vi "总控程序 _2026.vi"() -> ()   [LabVIEW 2026]
uses:
  Supports/CSM Names.ctl
  Supports/sPanel Data.ctl
  <userlib>/_NEVSTOP/Communicable State Machine(CSM)/_Polymophic/CSM - Filter Duplicated Lines.vi
  76f8fc9d-696a-4ccc-8dd7-48bdb3d8b640.vi
  bb814cf8-2670-4bb2-81f9-09f44a02b01b.vi
  fcea05e1-ee31-4bad-8a55-4c21f91279eb.vi
  86c0e0eb-f419-4f98-b770-132e8c8a6837.vi
  4aaf4cac-01b3-4f48-b7c2-c419dc6ea011.vi
  6f23f83d-c4e9-4f99-a0e1-96770a8349f6.vi
  8f3727b1-d436-4491-a02b-c19b6576eb4a.vi
  3b795a98-2c3e-48b2-8c77-c6d72b6bb2f2.vi
  a3e68da9-8157-4524-98c0-5afabb5447f5.vi
  436c64fb-213b-48d1-93d7-30f6f7eef33b.vi
  86e951a0-9aaf-40ac-b60e-6206b3d1b492.vi
  <userlib>/_NEVSTOP/Communicable State Machine(CSM)/_Polymophic/CSM - Replace Marks in Messages.vi
  29ebbcbd-9bba-4aa0-9480-6c7032d08e2a.vi
  31245a41-a78f-4281-aa79-3581d5ea05b1.vi
  ac877760-a0f7-42e3-86ce-81130eb57136.vi
  bb062149-d510-40e2-9bfa-d104bbeea636.vi
  <userlib>/_NEVSTOP/Communicable State Machine(CSM)/AdvanceAPI/CSM - Compact Multiple States.vi
  <userlib>/_NEVSTOP/Communicable State Machine(CSM)/AdvanceAPI/CSM - Break Down Multiple States String.vi
  <userlib>/_NEVSTOP/Communicable State Machine(CSM)/_Shared/Remove Comments from Single-line.vi
  <userlib>/_NEVSTOP/Communicable State Machine(CSM)/_Shared/Split Single-line Message.vi
  <userlib>/_NEVSTOP/Communicable State Machine(CSM)/_Shared/Trim Single-line Text.vi
  <userlib>/_NEVSTOP/Communicable State Machine(CSM)/AdvanceAPI/CSM - Revert Arguments-Safe String.vi
  <userlib>/_NEVSTOP/Communicable State Machine(CSM)/AdvanceAPI/CSM - Make String Arguments Safe.vi
  <userlib>/_NEVSTOP/Communicable State Machine(CSM)/AdvanceAPI/CSM - Keywords.vi
  <userlib>/_NEVSTOP/Communicable State Machine(CSM)/addons/API-String-Arugments-Support/_Support/Data To API String Arguments.vi
  <userlib>/_NEVSTOP/Communicable State Machine(CSM)/addons/INI-Static-Variable-Support/_Support/instances/_CSM - Read File Logger Configuration - v1.0.vi
  <userlib>/_NEVSTOP/Communicable State Machine(CSM)/addons/API-String-Arugments-Support/_Support/Convert API String Arguments to Data(variant).vi
  <userlib>/_NEVSTOP/Communicable State Machine(CSM)/Communicable State Machine.lvlib
  <userlib>/_NEVSTOP/Communicable State Machine(CSM)/addons/MassData-Parameter/CSM MassData Parameter Support.lvlib
  <userlib>/_NEVSTOP/Communicable State Machine(CSM)/addons/INI-Static-Variable-Support/INI-Static-Variable-Support.lvlib
  <userlib>/_NEVSTOP/Communicable State Machine(CSM)/addons/Watchdog/CSM Watchdog.lvlib
  <userlib>/_NEVSTOP/Communicable State Machine(CSM)/addons/Logger/CSM File Logger.lvlib
panel:
  in  "DS1":bool
  in  "HM1":bool
  in  "MO2":bool
  in  "MO1":bool
  in  "ZO1":bool
  in  "PS2":bool
  in  "PS1":bool
  in  "WK2":bool
  in  "P3-C3开关":bool
  in  "P3-C2开关":bool
  in  "P2-C3开关":bool
  in  "P2-C2开关":bool
  in  "P1-C3开关":bool
  in  "P1-C2开关":bool
  in  "WK1":bool
  in  "TP2":bool
  in  "TP1":bool
  in  "OP3":bool
  in  "OP2":bool
  in  "OP1":bool
  in  "停止":bool
  in  "波形查看":T1(tab)
  in  "合并保存？":bool
  in  "温度数据保存文件-时间":string
  in  "CSM Name":string="CSM-Module"
  out "State History":string
  out "Error Occurred":errorcluster
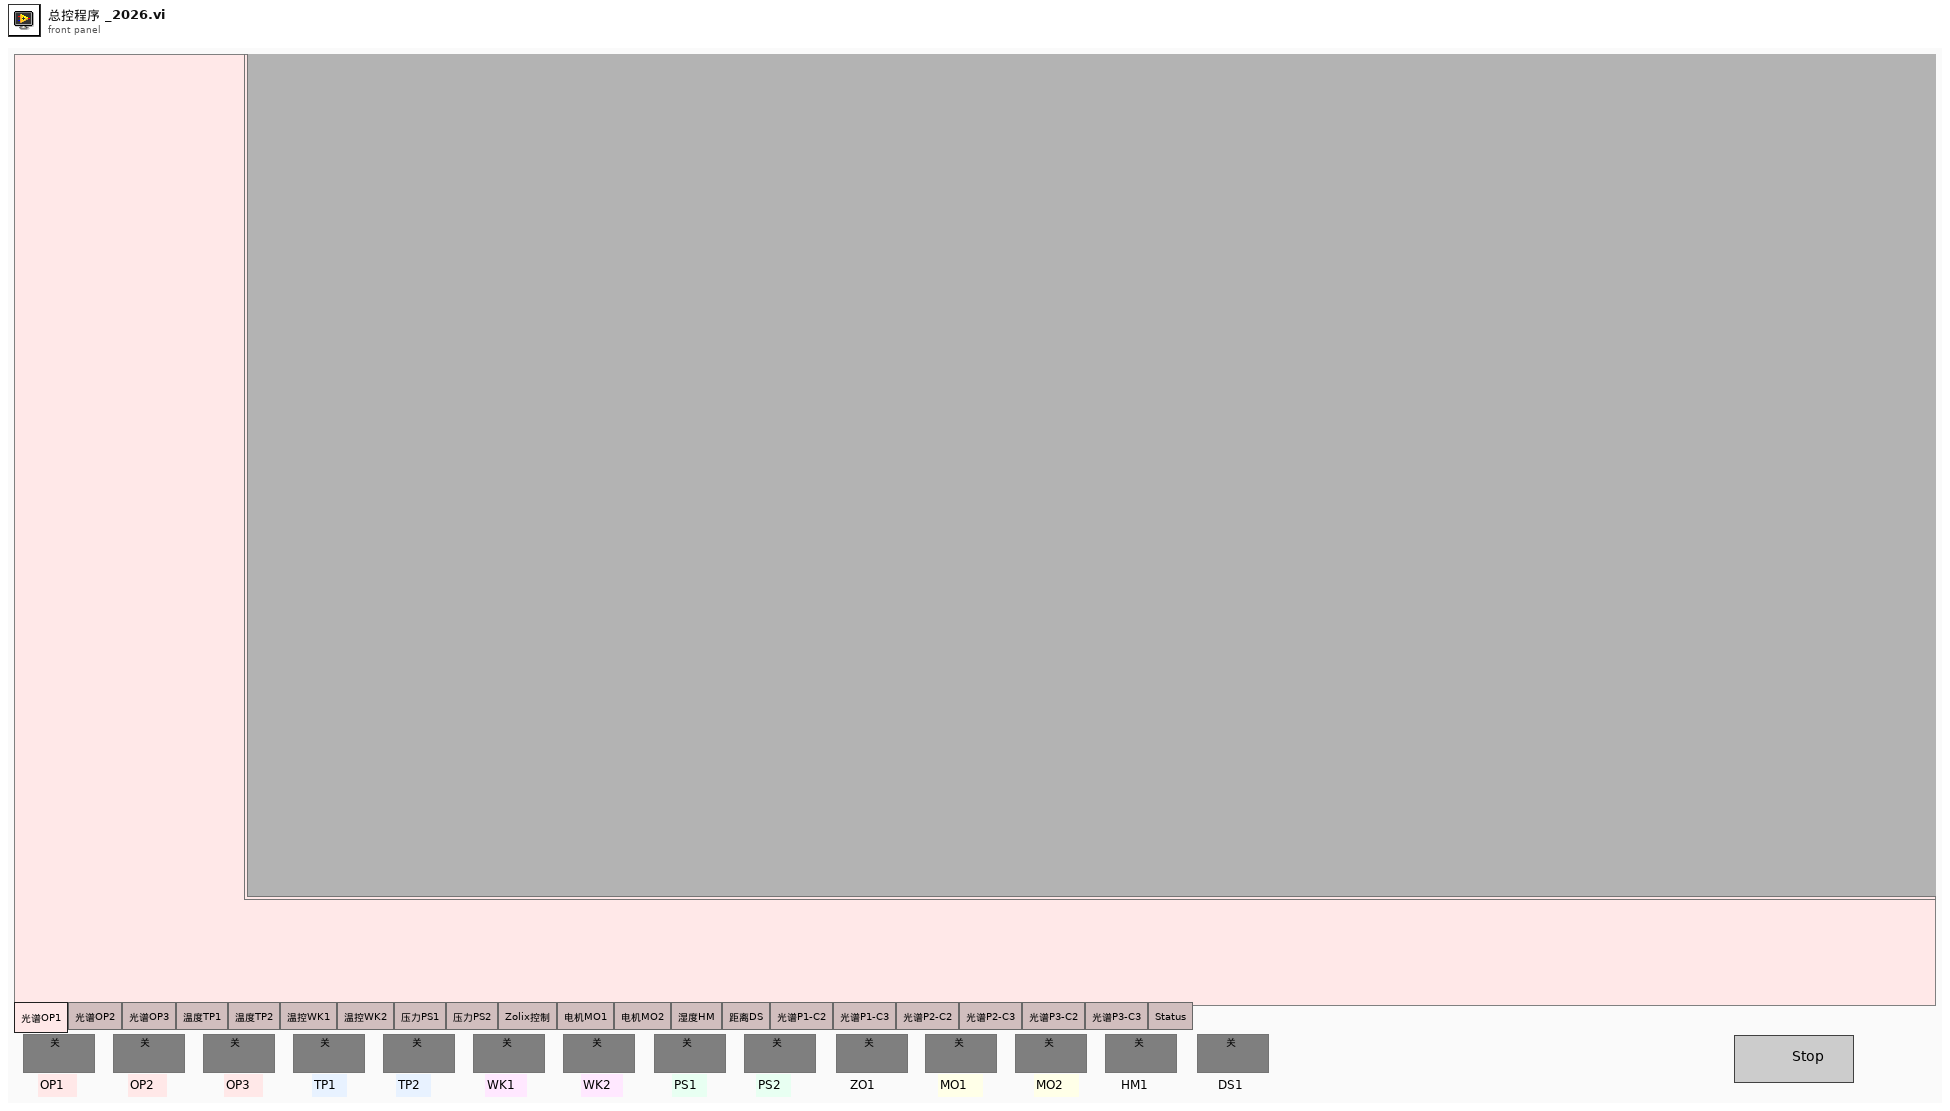
[diagram p1: front panel]
types:
  T1 = enum32{"光谱OP1", "光谱OP2", "光谱OP3", "温度TP1", "温度TP2", "温控WK1", "温控WK2", "压力PS1", "压力PS2", "Zolix控制", "电机MO1", "电机MO2", "湿度HM", "距离DS", "光谱P1-C2", "光谱P1-C3", "光谱P2-C2", "光谱P2-C3", "光谱P3-C2", "光谱P3-C3", "Status"}
  T2 = cluster{"Enable":bool, "Limit":cluster{"FileSize":i64, "FileNum":i32}, "Timestamp.Format":string, "AutoExit":bool}
  T3 = enum32{"Invalid", "Standard", "Closed", "Hidden", "Minimized", "Maximized"}
  T4 = enum32{"invalid app kind", "Development System", "Run Time System", "Student Edition", "Embedded LabVIEW", "Evaluation", "Custom"}
  T5 = typedef "sPanel Data.ctl" = cluster{"子面板":refnum<vi>, "程序引用":refnum<vi>, "CSM Name":string}
  T6 = typedef "温度保存信息.ctl" = cluster{"温度保存-时间":string, "合并保存？":bool, "保存路径":path, "Intervals":dbl}
  T7 = typedef "Communicable State Machine.lvlib/_CSM_Response Source Message.ctl" = cluster{"‘State":string, "’Arguments":string, "’Error":errorcluster}
  T8 = cluster{"Current VI Reference":refnum<vi>, "Close Panel on Exit?":bool}
  T9 = typedef "CSM Names.ctl" = string[]
  T10 = cluster{"Core":cluster{"Current VI Reference":refnum<vi>, "Close Panel on Exit?":bool}, "索引汇总":cluster{"子面板索引":refnum<vi>[], "程序索引":refnum<vi>[], "CSM Names":T9, "开关索引":refnum<vi>[]}, "Data Save":bool, "Stop":bool}
  T11 = cluster{"子面板索引":refnum<vi>[], "程序索引":refnum<vi>[], "CSM Names":T9, "开关索引":refnum<vi>[]}
  T12 = cluster{"子面板HM1":refnum<vi>, refnum<vi>, "CSM Name":string}
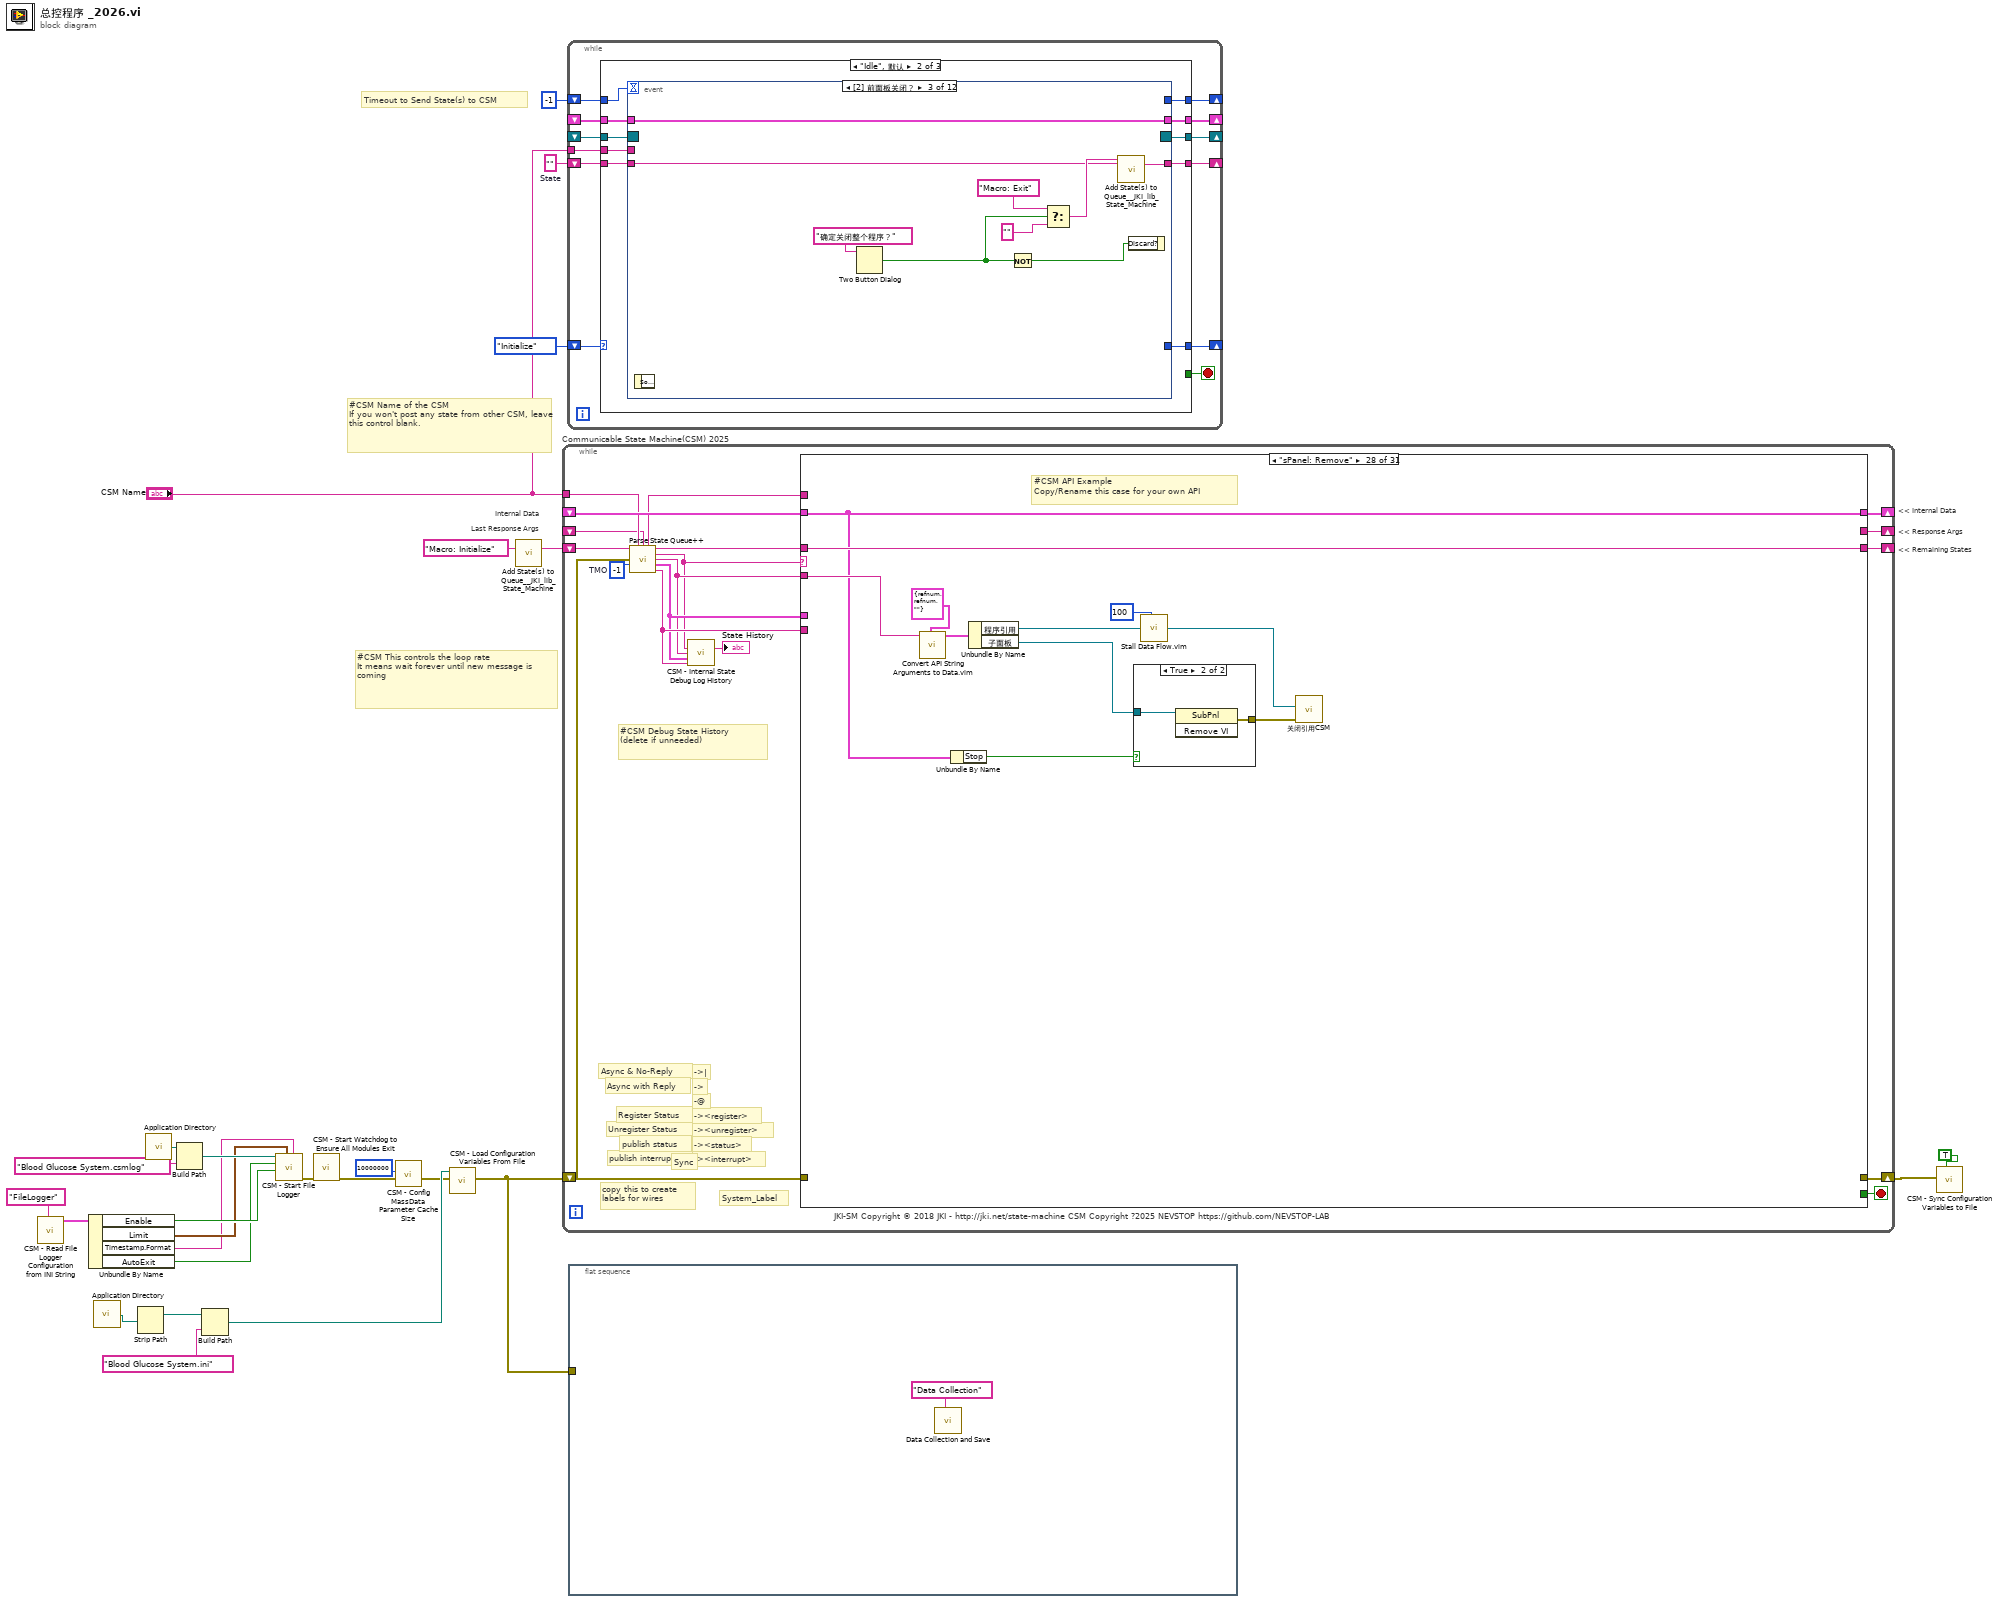
[diagram p0: block diagram]
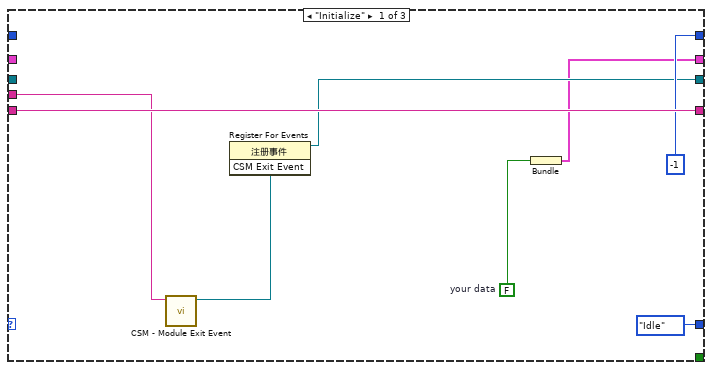
[diagram p2: hidden frame]
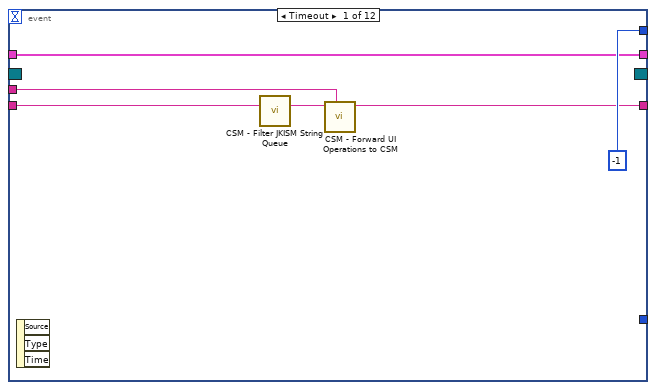
[diagram p3: hidden frame]
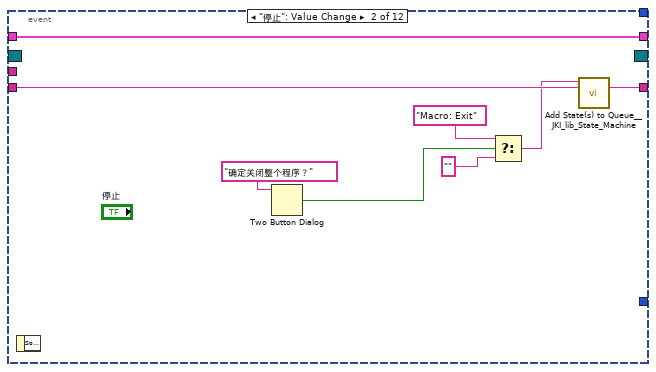
[diagram p4: hidden frame]
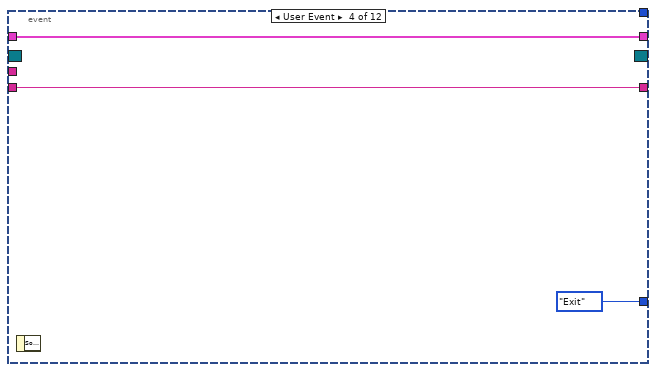
[diagram p5: hidden frame]
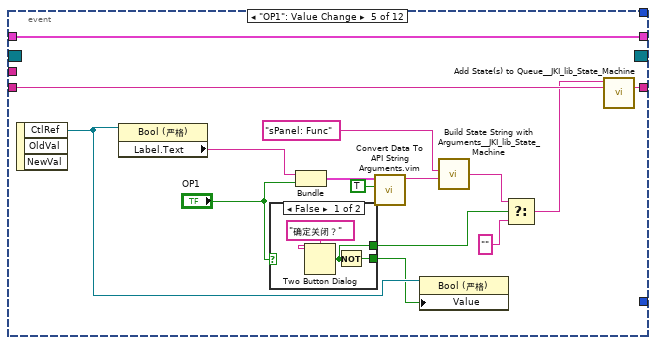
[diagram p6: hidden frame]
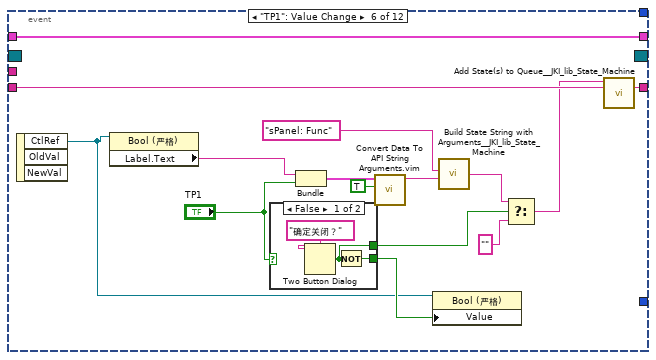
[diagram p8: hidden frame]
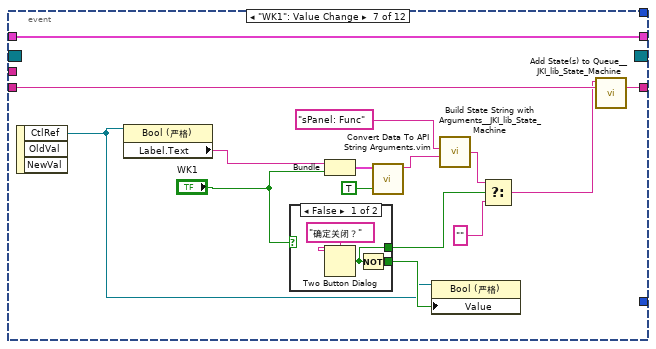
[diagram p10: hidden frame]
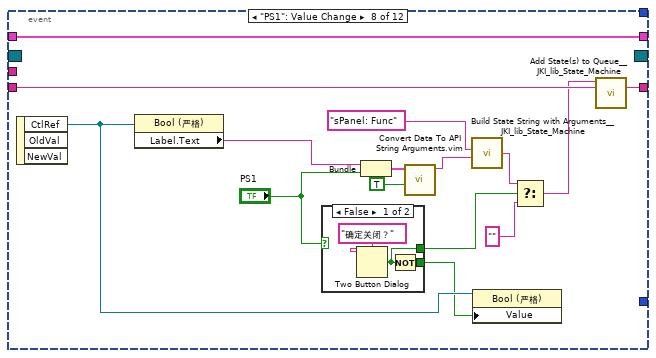
[diagram p12: hidden frame]
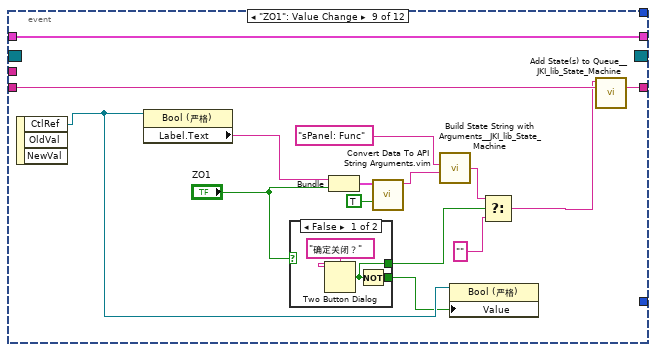
[diagram p14: hidden frame]
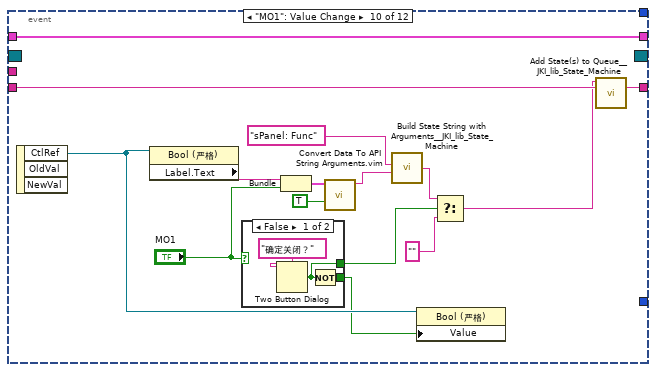
[diagram p16: hidden frame]
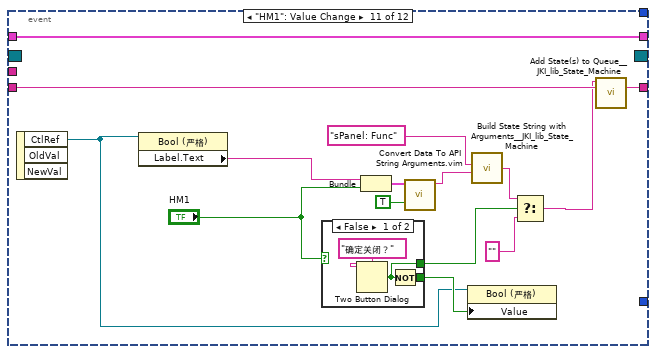
[diagram p18: hidden frame]
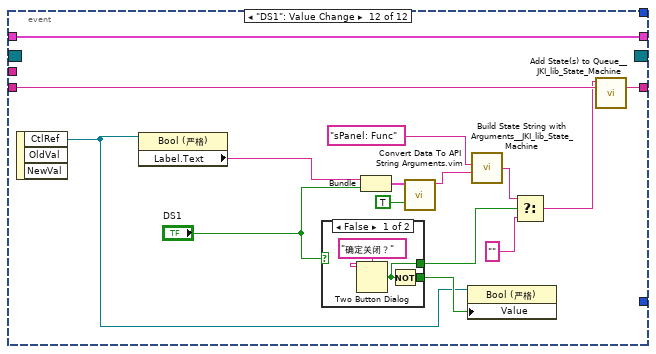
[diagram p20: hidden frame]
diagram:
  w25 = ""  # State
  # "Timeout to Send State(s) to CSM"
  # "Last Response Args"
  # "Internal Data"
  # "#CSM Name of the CSM\nIf you won't post any state from other CSM, leave this control blank."
  # "#CSM This controls the loop rate\nIt means wait forever until new message is coming"
  # "<< Internal Data"
  # "<< Response Args"
  # "<< Remaining States"
  n1 = call-poly <userlib>:"CSM - Read File Logger Configuration from INI String.vi"("Section Name(\"FileLogger\")"="FileLogger" ("Section Name(\"\" as Default)")) -> ("FileLogger Configuration-v1"=w14:T2)  [unwired: 7 in, 1 out]
  n2 = Unbundle By Name(w14) -> ("Enable"=w13:bool, "Limit"=w12:cluster{"FileSize":i64, "FileNum":i32}, "Timestamp.Format"=w10:string, "AutoExit"=w11:bool)
  n3 = call <vilib>:"Application Directory.vi"() -> ("Application Directory"=w6:path)
  n4 = Strip Path(path=w6) -> (stripped path=w5:path)  [unwired: 1 out]
  n5 = call <vilib>:"Application Directory.vi"() -> ("Application Directory"=w19:path)
  n6 = Build Path(base path=w19, name or relative path="Blood Glucose System.csmlog") -> (appended path=w17:path)
  n7 = Build Path(base path=w5, name or relative path="Blood Glucose System.ini") -> (appended path=w3:path)
  n8 = call <userlib>:"CSM - Start File Logger.vi"("Timestamp Format"=w10, "Log Limit"=w12, "Watchdog? (T)"=w13, "Exit When All Module Exist? (F)"=w11, "Log File Path"=w17) -> ("error out"=w16:errorcluster)  [unwired: 4 in, 2 out]
  n9 = call <userlib>:"CSM - Start Watchdog to Ensure All Modules Exit.vi"("error in (no error)"=w16) -> ("error out"=w20:errorcluster)  [unwired: 10 in]
  n10 = call <userlib>:"CSM - Config MassData Parameter Cache Size.vi"("Error in"=w20, "Size (50M)"=10000000 ("size(1M)")) -> ("Error out"=w2:errorcluster)  [unwired: 9 in]
  n11 = call <userlib>:"CSM - Load Configuration Variables From File.vi"("error in (no error)"=w2, "Configuration Path"=w3) -> ("error out"=w1:errorcluster)  [unwired: 7 in]
  n12 = call <vilib>:"Add State(s) to Queue__JKI_lib_State_Machine.vi"("State(s) in (\"\")"="Macro: Initialize" ("Init State(\"Macro: Initialize\")")) -> ("States Out"=w22:string)  [unwired: 14 in]
  n13 = while "Communicable State Machine(CSM) 2025" {
    shift-right: [w39] -> _
    shift-left: _ -> [w38]
    shift-right: [w42] -> w7
    shift-left: w1 -> [w28]
    shift-right: [w41] -> _
    shift-left: w22 -> [w43]
    tunnel: "CSM Name" -> [w35]
    shift-right: [w36] -> _
    shift-left: _ -> [w30]
    stop <- w40 stop-if-true
    w37 = -1  # TMO
    # "#CSM Debug State History\n(delete if unneeded)"
    # "-><interrupt>"
    # "-><status>"
    # "-><unregister>"
    # "-><register>"
    # "-@"
    # "->"
    # "->|"
    # "publish interrupt"
    # "publish status"
    # "Unregister Status"
    # "Register Status"
    # "Sync"
    # "Async with Reply"
    # "Async & No-Reply"
    # "JKI-SM Copyright © 2018 JKI - http://jki.net/state-machine CSM Copyright ?2025 NEVSTOP https://github.com/NEVSTOP-LAB"
    # "copy this to create labels for wires"
    # "System_Label"
    n14 = call <userlib>:"Parse State Queue++.vi"("State Queue"=w43, "Name (\"\" to Use UUID)"=w35, "Response Arguments"=w30, "Previous Error"=w28, "Dequeue (1 ms)"=w37) -> ("Name Used"=w29:string, "Remaining States"=w44:string, "Current State"=w31:string, "Arguments"=w32:string, "Additional Information"=w33:T7, "Source CSM"=w34:string)  [unwired: 5 in]
    n15 = call <userlib>:"CSM - Internal State Debug Log History.vi"("State"=w31, "Arguments (\"\")"=w32, ">> Response Source Message >>"=w33, "Source (\"\")"=w34) -> ("Debug Log"=→"State History":string)  [unwired: 11 in]
    n16 = case shown="\"sPanel: Remove\"" w31 {
      selector: w31 -> [_ _ _ w55 _ _ _ _ _ _ _ _ _ _ _ _ _ _ _ _ _ _ _ _ _ _ _ _ _ _ _]
      tunnel: w44 -> [w45 w48 w51 w59 w64 w70 w95 w101 w107 w117 w130 w142 w146 w149 w199 w201 w207 w210 w216 w221 w225 w232 w243 w245 w275 w294 w317 w331 w334 w342 w378]
      tunnel: w32 -> [_ _ _ _ _ w69 w91 w98 w104 w112 _ _ _ _ _ _ _ _ _ _ _ _ _ _ w277 w292 w309 w327 _ _ _]
      tunnel: w38 -> [w46 w47 w49 w57 w63 w75 w93 w99 w105 w115 w129 w136 w144 w147 _ w200 w202 w208 w211 w219 w223 w227 w237 w244 w272 w296 w319 w324 w336 w339 w360]
      tunnel: [_ _ _ w52 w65 errorcluster {"status"=FALSE, "code"=0, "source"=""} ("error out") w88 w96 w102 w118 _ _ _ _ _ _ w203 _ _ _ _ w234 _ _ w279 _ w320 _ w337 w344 w380] -> w42
      tunnel: w28 -> [_ _ _ w53 w65 w73 w89 w97 w103 _ _ _ _ _ _ _ w204 _ _ _ _ w234 _ _ w279 _ w320 _ w337 w344 w380]
      tunnel: [w45 w48 w50 w58 w64 w71 w94 w100 w106 w116 w130 w141 w145 w148 w198 w201 w206 w209 w215 w220 w224 w233 w242 w245 w276 w295 w318 w331 w335 w343 w379] -> w41
      tunnel: [_ _ _ _ _ _ TRUE _ _ _ _ _ TRUE _ _ _ _ _ _ _ _ _ _ _ _ _ _ _ _ _ _] -> w40
      tunnel: [w46 w47 w49 w57 w63 w75 w93 w99 w105 w114 w129 w140 w144 w147 w197 w200 w202 w208 w211 w219 w223 w227 w235 w244 w272 w296 w319 w324 w336 w338 w359] -> w39
      tunnel: w34 -> [_ _ _ _ _ w68 _ _ _ w108 _ _ _ _ _ _ _ _ _ _ _ _ _ _ _ _ _ _ _ _ _]
      tunnel: w33 -> [_ _ _ _ _ w67 _ _ _ w113 _ _ _ _ _ _ _ _ _ _ _ _ _ _ _ _ _ _ _ _ _]
      tunnel: [_ _ _ "" w60 _ _ _ _ _ _ _ _ _ _ _ _ _ _ _ _ _ _ _ _ _ _ _ _ _ _] -> w36
      tunnel: w29 -> [_ _ _ w54 _ _ w90 _ _ _ _ _ _ _ _ _ _ _ _ _ _ _ _ _ _ _ _ _ _ _ _]
      frame "", "Idle" {
        # "#CSM \"Idle/Event Handler\"\nexecutes when the state queue is empty"
      }
      frame "CSM Documentation" {
        # "#CSM State Syntax\n\n// Comment line, all text to the right of “//” will be ignored\n// Local Message Example\nDoSth: DoA >> Arguments\n\n// Sync Call Example\nAPI: xxxx >> Arguments -@ TargetModule\n\n// Async Call Example\nAPI: xxxx >> Arguments -> TargetModule\n\n// Async Call without Reply Example\nAPI: xxxx >> Arguments ->| TargetModule\n\n// Broadcast normal status:\nStatus >> StatusArguments  -><status>\n\n// Broadcast Interrupt status:\nInterrupt >> StatusArguments  -><interrupt>\n\n// Register Source Module's status to Handler Module\nStatus@Source Module >> Handler Module@Handler Module -><register>\n\n// Unegister Source Module's status\nStatus@Source Module >> Handler Module -><unregister>"
        # "#CSM README FIRST\n\nCommunicable State Machine(CSM) is a LabVIEW application framework that builds upon JKI State Machine(JKISM). It follows the pattern of JKISM and extends the keywords to describe message communication between modules, including concepts such as Sync-Message, Async-Message, Subscription/Unsubscription of status - essential elements for creating reusable code modules. For more information, please visit the CSM wiki: https://nevstop-lab.github.io/CSM-Wiki/\n\nFor instructions on JKI State Machine, visit: \n    http://jki.net/state-machine/\nFor information about CSM, visit: \n    https://github.com/NEVSTOP-LAB"
        # "#CSM \"Documentation\"\nCase for holding CSM Documenation"
      }
      frame "---------- Core ----------" {
        # "#CSM \"Category Seperator\"\nDo not put any code in this frame."
        n17 = call <vilib>:"Add State(s) to Queue__JKI_lib_State_Machine.vi"("State(s) in (\"\")"=w51) -> ("States Out"=w50:string)  [unwired: 14 in]
      }
      frame Default {
        # "#CSM \"Default\"\nthis is used to capture unhandled states and typos"
        n18 = call <userlib>:"CSM Unhandled State Error.vi"("error in (no error)"=w53, "Undefined State"=w55, "CSM Name"=w54) -> ("error out"=w52:errorcluster)  [unwired: 8 in]
        n19 = call <vilib>:"Add State(s) to Queue__JKI_lib_State_Machine.vi"("State(s) in (\"\")"=w59) -> ("States Out"=w58:string)  [unwired: 14 in]
      }
      frame "VI Reference" {
        n20 = Unbundle By Name(w63) -> ("Core"=w62:T8)
        n21 = Unbundle By Name(w62) -> ("Current VI Reference"=w61:refnum<vi>)
        n22 = call <userlib>:"CSM - Convert Data to HexStr.vi"("Variant"=w61) -> ("HEX String (0-9,A-F)"=w60:string)  [unwired: 8 in]
      }
      frame "Error Handler" {
        # "#CSM \"Error Handler\"\nYou can also output any states to clean-up after errors occur"
        # "Clear error"
        n23 = case shown="错误" w73 {
          selector: w73 -> [_ w82]
          tunnel: [w80 w84] -> w72
          tunnel: w70 -> [w80 w83]
          tunnel: w69 -> [w79 _]
          tunnel: w68 -> [_ _]
          tunnel: w67 -> [_ _]
          tunnel: [w77 w82] -> w66
          frame No Error {
            n24 = call <userlib>:"CSM - Convert Argument to Error.vi"("Argument"=w79) -> ("Error"=w78:errorcluster)  [unwired: 4 in]
            n25 = flat-sequence {
              tunnel: w78 -> [w81]
              tunnel: [w81] -> w77
              frame #0 {
                # "#CSM External Error Handler Case\nUsually, it's because This CSM register others' \"Error Occurred\" status with \"Error Handler\". If other CSM have any error, the error will be passed here for central handling."
              }
            }
          }
          frame Error {
            # "#CSM Internal Error Handler Case \nIf any error Occurred, \"Error Occurred\" \nstatus update will be broadcasted to system.\nParameter is Error Cluster."
            n26 = call <userlib>:"CSM - Convert Error to Argument.vi"("Error"=w82) -> ("Argument"=w86:string)  [unwired: 4 in]
            n27 = call <vilib>:"Build State String with Arguments__JKI_lib_State_Machine.vi"("Arguments (\"\")"=w86, "State"="Error Occurred" ("Status with Arguments")) -> ("State with Arguments"=w85:string)  [unwired: 4 in]
            n28 = call <userlib>:"CSM - Broadcast Status Change.vi"("Status With Arguments"=w85, "State Queue"=w83) -> ("Remaining States"=w84:string)  [unwired: 13 in]
          }
        }
        "Error Occurred" <- w66
        n29 = call <vilib>:"Add State(s) to Queue__JKI_lib_State_Machine.vi"("State(s) in Front (\"\")"="// Post Error States", "State(s) in (\"\")"=w72) -> ("States Out"=w71:string)  [unwired: 13 in]
      }
      frame "Critical Error" {
        # "#CSM \"Critical Error\"\nWhen any un-recoverable error occurs, CSM goes into this case."
        # "#CSM Stop in Critical Error\nWhen Critical Error occurs, Stop the loop immediately. Do NOT change this unless you fully understand the impact."
        n30 = call <userlib>:"CSM Critical Error.vi"("error in (no error)"=w89, "Arugments (As Reason)"=w91, "CSM Name"=w90) -> ("error out"=w88:errorcluster)  [unwired: 8 in]
        n31 = call <vilib>:"Add State(s) to Queue__JKI_lib_State_Machine.vi"("State(s) in (\"\")"=w95) -> ("States Out"=w94:string)  [unwired: 14 in]
      }
      frame "Target Timeout Error" {
        # "#CSM \"Target Timeout Error\"\nWhen This CSM could not get the sync-call response in time, This CSM goes into this case."
        n32 = call <userlib>:"CSM Target Timeout Error.vi"("error in (no error)"=w97, "Arguments (As CSM Name)"=w98) -> ("error out"=w96:errorcluster)  [unwired: 9 in]
        n33 = call <vilib>:"Add State(s) to Queue__JKI_lib_State_Machine.vi"("State(s) in (\"\")"=w101) -> ("States Out"=w100:string)  [unwired: 14 in]
      }
      frame "Target Error" {
        # "#CSM \"Target Error\"\nWhen This CSM try to communicate with an un-existed CSM, This CSM goes into this case."
        n34 = call <userlib>:"CSM Target Error.vi"("error in (no error)"=w103, "Arguments (As CSM Name)"=w104) -> ("error out"=w102:errorcluster)  [unwired: 9 in]
        n35 = call <vilib>:"Add State(s) to Queue__JKI_lib_State_Machine.vi"("State(s) in (\"\")"=w107) -> ("States Out"=w106:string)  [unwired: 14 in]
      }
      frame "Async Response", "Response" {
        n36 = Unbundle(w113) -> ("‘State"=w109:string, "’Arguments"=w111:string, "’Error"=w110:errorcluster)
        n37 = case shown="\"Data Collection\"" w108 {
          tunnel: [w119 w127] -> w116
          tunnel: w117 -> [w120 w127]
          tunnel: [w122 w126] -> w114
          tunnel: w115 -> [w122 w126]
          tunnel: [w121 w125] -> w118
          tunnel: w110 -> [w121 w125]
          tunnel: w112 -> [_ w124]
          tunnel: w111 -> [_ _]
          tunnel: w109 -> [_ w123]
          frame Default {
            # "#CSM \"Async Response\"\nHandle Async-call Response (\"Async Response\" for ->)"
            # "#CSM \"Response\"\nHandle Sync-call Response (\"Response\" for -@)"
            # "#CSM Response Comments\nAfter Message is executed, CSM goes to this state for receive the response.\n    For Async Message(->), \"Async Response\" is used. This CSM will goes to \"Async Message Posted\" immediately and receive the \"Async Response\" after the callee finishes the message.\n    For Sync Message(@),  This CSM will wait until the message is done and immediately goes to \"Response\""
            n38 = call <vilib>:"Add State(s) to Queue__JKI_lib_State_Machine.vi"("State(s) in (\"\")"=w120) -> ("States Out"=w119:string)  [unwired: 14 in]
          }
          frame "Data Collection" {
            n39 = case shown="\"API: Start\"" w123 {
              tunnel: w124 -> [_ w128]
              frame "假", Default {
              }
              frame "API: Start" {
                n40 = local write "温度数据保存文件-时间"(w128) -> ()
              }
            }
          }
        }
      }
      frame "Async Message Posted" {
        # "#CSM \"Async Message Posted\"\nAfter Async Message is posted (-> or ->| ), CSM goes to this state for post-action.\nYou can use Argument - State to tell which Async Message is called."
      }
      frame "Initialize Core Data" {
        # "#CSM \"Initialize Core Data\"\nThis is used to determine panel behavior on exit"
        # "originally closed?"
        # "exe?"
        # "If panel starts closed or is an EXE, then close it when we exit"
        n41 = property class="VI"() -> ("FP.State"=w133:T3)  [unwired: 2 in, 2 out]
        n42 = property class="App"() -> ("App.Kind"=w139:T4)  [unwired: 2 in, 2 out]
        n43 = control-ref of="Current VI Reference"() -> (w134:refnum<vi>)
        n44 = Equal?(x=w133, y=T3."Closed" ("Front Panel Window:State")) -> (x = y?=w131:bool)
        n45 = Equal?(x=w139, y=T4."Run Time System" ("Application:Kind")) -> (x = y?=w137:bool)
        n46 = Or(x=w131, y=w137) -> (x .or. y?=w135:bool)
        n47 = Bundle By Name(cluster=w136, "Core.Current VI Reference"=w134, "Core.Close Panel on Exit?"=w135) -> (w140:T10)
        n48 = call <vilib>:"Add State(s) to Queue__JKI_lib_State_Machine.vi"("State(s) in (\"\")"=w142) -> ("States Out"=w141:string)  [unwired: 14 in]
      }
      frame "Exit" {
        # "#CSM \"Exit\"\nCase for exiting the loop. No errors that occur here will be handled."
        n49 = call <vilib>:"Add State(s) to Queue__JKI_lib_State_Machine.vi"("State(s) in (\"\")"=w146) -> ("States Out"=w145:string)  [unwired: 14 in]
      }
      frame "---------- Data ----------" {
        # "#CSM \"Category Seperator\"\nDo not put any code in this frame."
        n50 = call <vilib>:"Add State(s) to Queue__JKI_lib_State_Machine.vi"("State(s) in (\"\")"=w149) -> ("States Out"=w148:string)  [unwired: 14 in]
      }
      frame "Data: Initialize" {
        w153 = FALSE  # Stop
        w154 = T11 {"子面板索引"=[], "程序索引"=[], "CSM Names"=[], "开关索引"=[]}  # 索引汇总
        w176 = FALSE  # Data Save
        w189 = T9 ["OP1", "TP1", "WK1", "PS1", "ZO1", "MO1", "HM1", "DS1"]  # CSM Names
        w196 = T8 {"Current VI Reference"=refnum, "Close Panel on Exit?"=FALSE}  # Core
        # "子面板添加\n程序引用添加\nCSMname添加\n布尔控件引用调整\n布尔控件事件设置"
        # "#CSM \"Data: Initialize\"\nInitialize the shift-register data, here.\n(data names are defined by what you wire into the bundle function)"
        # "#CSM Data names and types of shift register data are defined by this bundle."
        n51 = control-ref of="子面板DS1"() -> (w151:refnum<vi>)
        n52 = control-ref of="DS1"() -> (w150:refnum<vi>)
        n53 = control-ref of="TP1"() -> (w179:refnum<vi>)
        n54 = control-ref of="WK1"() -> (w177:refnum<vi>)
        n55 = control-ref of="PS1"() -> (w174:refnum<vi>)
        n56 = control-ref of="ZO1"() -> (w169:refnum<vi>)
        n57 = control-ref of="MO1"() -> (w168:refnum<vi>)
        n58 = control-ref of="HM1"() -> (w167:refnum<vi>)
        n59 = control-ref of="TP2"() -> (w166:refnum<vi>)
        n60 = control-ref of="WK2"() -> (w165:refnum<vi>)
        n61 = control-ref of="PS2"() -> (w164:refnum<vi>)
        n62 = control-ref of="MO2"() -> (w163:refnum<vi>)
        n63 = control-ref of="子面板HM1"() -> (w159:refnum<vi>)
        n64 = control-ref of="子面板MO1"() -> (w160:refnum<vi>)
        n65 = Build Array(w179, w177, w174, w169, w168, w167, w150, w166, w165, w164, w163) -> (w172:refnum<vi>[])
        n66 = control-ref of="子面板ZO1"() -> (w161:refnum<vi>)
        n67 = vi-ref "UI-距离测量.lvlib:距离测量 - DS.vi"() -> (w152:refnum<vi>)
        n68 = vi-ref "UI-湿度测量.lvlib:湿度测量 - HM1.vi"() -> (w155:refnum<vi>)
        n69 = control-ref of="子面板PS1"() -> (w175:refnum<vi>)
        n70 = control-ref of="OP1"() -> (w170:refnum<vi>)
        n71 = vi-ref "UI-步进.lvlib:步进电机 - MO1.vi"() -> (w156:refnum<vi>)
        n72 = control-ref of="OP2"() -> (w180:refnum<vi>)
        n73 = control-ref of="OP3"() -> (w181:refnum<vi>)
        n74 = control-ref of="P1-C2开关"() -> (w182:refnum<vi>)
        n75 = control-ref of="P1-C3开关"() -> (w183:refnum<vi>)
        n76 = control-ref of="P2-C2开关"() -> (w184:refnum<vi>)
        n77 = control-ref of="P2-C3开关"() -> (w185:refnum<vi>)
        n78 = control-ref of="P3-C2开关"() -> (w186:refnum<vi>)
        n79 = control-ref of="P3-C3开关"() -> (w187:refnum<vi>)
        n80 = control-ref of="子面板WK1"() -> (w195:refnum<vi>)
        n81 = vi-ref "UI-Zolix.lvlib:Zolix控制 - ZO1.vi"() -> (w157:refnum<vi>)
        n82 = Build Array(w180, w181, w182, w183, w184, w185, w186, w187) -> (w171:refnum<vi>[])
        n83 = vi-ref "UI-压力.lvlib:压力测量 - PS1.vi"() -> (w173:refnum<vi>)
        n84 = control-ref of="子面板TP1"() -> (w194:refnum<vi>)
        n85 = vi-ref "UI-温度控制.lvlib:温度控制 - WK1.vi"() -> (w192:refnum<vi>)
        n86 = control-ref of="子面板 - OP1"() -> (w162:refnum<vi>)
        n87 = Build Array (concatenate)(w170, w172, w171) -> (w178:refnum<vi>[])
        n88 = vi-ref "UI-温度采集.lvlib:温度采集 - TP1.vi"() -> (w193:refnum<vi>)
        n89 = vi-ref "UI-无创.lvlib:无创血糖测量 - OP1.vi"() -> (w158:refnum<vi>)
        n90 = Build Array(w162, w194, w195, w175, w161, w160, w159, w151) -> (w191:refnum<vi>[])
        n91 = Build Array(w158, w193, w192, w173, w157, w156, w155, w152) -> (w190:refnum<vi>[])
        n92 = Bundle(cluster=w154, "子面板索引"=w191, "程序索引"=w190, "CSM Names"=w189, "开关索引"=w178) -> (w188:T11)
        n93 = Bundle("Core"=w196, "索引汇总"=w188, "Data Save"=w176, "Stop"=w153) -> (w197:T10)  [unwired: 1 in]
        n94 = call <vilib>:"Add State(s) to Queue__JKI_lib_State_Machine.vi"("State(s) in (\"\")"=w199) -> ("States Out"=w198:string)  [unwired: 14 in]
      }
      frame "Data: Update Indicators" {
        n95 = control-ref of="OP1"() -> ()  [unwired: 1 out]
        n96 = control-ref of="OP2"() -> ()  [unwired: 1 out]
        n97 = control-ref of="OP3"() -> ()  [unwired: 1 out]
        n98 = control-ref of="P1-C2开关"() -> ()  [unwired: 1 out]
        n99 = control-ref of="P1-C3开关"() -> ()  [unwired: 1 out]
        n100 = control-ref of="P2-C2开关"() -> ()  [unwired: 1 out]
        n101 = control-ref of="P2-C3开关"() -> ()  [unwired: 1 out]
        n102 = control-ref of="P3-C2开关"() -> ()  [unwired: 1 out]
        n103 = control-ref of="P3-C3开关"() -> ()  [unwired: 1 out]
        n104 = control-ref of="TP1"() -> ()  [unwired: 1 out]
        n105 = control-ref of="TP2"() -> ()  [unwired: 1 out]
        n106 = control-ref of="WK1"() -> ()  [unwired: 1 out]
        n107 = control-ref of="WK2"() -> ()  [unwired: 1 out]
        n108 = control-ref of="PS1"() -> ()  [unwired: 1 out]
        n109 = control-ref of="PS2"() -> ()  [unwired: 1 out]
        n110 = control-ref of="MO1"() -> ()  [unwired: 1 out]
        n111 = control-ref of="MO2"() -> ()  [unwired: 1 out]
        n112 = control-ref of="ZO1"() -> ()  [unwired: 1 out]
        n113 = control-ref of="HM1"() -> ()  [unwired: 1 out]
        n114 = control-ref of="DS1"() -> ()  [unwired: 1 out]
        n115 = control-ref of="子面板 - OP2"() -> ()  [unwired: 1 out]
        n116 = control-ref of="子面板 - OP3"() -> ()  [unwired: 1 out]
        n117 = control-ref of="子面板 - P1 - C2"() -> ()  [unwired: 1 out]
        n118 = control-ref of="子面板 - P1 - C3"() -> ()  [unwired: 1 out]
        n119 = control-ref of="子面板 - P2 - C2"() -> ()  [unwired: 1 out]
        n120 = control-ref of="子面板 - P2 - C3"() -> ()  [unwired: 1 out]
        n121 = control-ref of="子面板 - P3 - C2"() -> ()  [unwired: 1 out]
        n122 = control-ref of="子面板 - P3 - C3"() -> ()  [unwired: 1 out]
        n123 = control-ref of="子面板TP2"() -> ()  [unwired: 1 out]
        n124 = control-ref of="子面板WK2"() -> ()  [unwired: 1 out]
        n125 = control-ref of="子面板PS2"() -> ()  [unwired: 1 out]
        n126 = control-ref of="子面板MO2"() -> ()  [unwired: 1 out]
      }
      frame "Data: Cleanup" {
        # "#CSM \"Data: Cleanup\"\nCleanup any data and references, here.\n(this is called automatically, by the Macro: Exit)"
        n127 = Unbundle By Name(w202) -> ("Core.Current VI Reference"=w205:refnum<vi>)
        n128 = Close Reference(reference=w205, error in (no error)=w204) -> (error out=w203:errorcluster)
        n129 = call <vilib>:"Add State(s) to Queue__JKI_lib_State_Machine.vi"("State(s) in (\"\")"=w207) -> ("States Out"=w206:string)  [unwired: 14 in]
      }
      frame "---------- UI ----------" {
        # "#CSM \"Category Seperator\"\nDo not put any code in this frame."
        n130 = call <vilib>:"Add State(s) to Queue__JKI_lib_State_Machine.vi"("State(s) in (\"\")"=w210) -> ("States Out"=w209:string)  [unwired: 14 in]
      }
      frame "UI: Initialize" {
        # "#CSM \"Category Seperator\"\nDo not put any code in this frame."
        n131 = Unbundle By Name(w211) -> ("索引汇总.开关索引"=w213:refnum<vi>[])
        n132 = for {
          tunnel: w213 -> [w218] mode=indexing
          tunnel: FALSE -> [w217]
          n133 = property class="Bool (严格)"(reference=w218, "Value"=w217) -> ()  [unwired: 1 in, 2 out]
        }
        n134 = local write "Error Occurred"(errorcluster {"status"=FALSE, "code"=0, "source"=""} ("错误常量")) -> ()
        n135 = call <vilib>:"Add State(s) to Queue__JKI_lib_State_Machine.vi"("State(s) in (\"\")"=w216) -> ("States Out"=w215:string)  [unwired: 14 in]
      }
      frame "---------- Macro ----------" {
        # "#CSM \"Category Seperator\"\nDo not put any code in this frame."
        n136 = call <vilib>:"Add State(s) to Queue__JKI_lib_State_Machine.vi"("State(s) in (\"\")"=w221) -> ("States Out"=w220:string)  [unwired: 14 in]
      }
      frame "Macro: Initialize" {
        # "#CSM \"Macro: Initialize\"\nInitialization Macro (This is called once, when the VI starts)"
        n137 = call <vilib>:"Add State(s) to Queue__JKI_lib_State_Machine.vi"("State(s) in Front (\"\")"="Data: Initialize\nInitialize Core Data\nData: Update Indicators\n\nUI: Initialize", "State(s) in (\"\")"=w225) -> ("States Out"=w224:string)  [unwired: 13 in]
      }
      frame "Macro: Exit Sub-Modules" {
        n138 = Unbundle By Name(w227) -> ("索引汇总.CSM Names"=w226:T9)
        n139 = call "CSMs2States.vi"("CSM Names"=w226, "States"="sPanel: Func") -> ("States Out"=w230:string)  [unwired: 9 in]
        n140 = call <vilib>:"Add State(s) to Queue__JKI_lib_State_Machine.vi"("State(s) in Front (\"\")"=w230, "State(s) in (\"\")"="Macro: Exit-@Data Collection\n") -> ("States Out"=w228:string)  [unwired: 13 in]
        n141 = call <vilib>:"Add State(s) to Queue__JKI_lib_State_Machine.vi"("State(s) in Front (\"\")"=w228, "State(s) in (\"\")"=w232) -> ("States Out"=w233:string)  [unwired: 13 in]
      }
      frame "Macro: Exit" {
        # "#CSM \"Macro: Exit\"\nExit Macro (This is called once, when the VI exits)"
        n142 = call <vilib>:"Add State(s) to Queue__JKI_lib_State_Machine.vi"("State(s) in Front (\"\")"="//Exit Sub-Modules ", "State(s) in (\"\")"="Macro: Exit Sub-Modules", "State(s) at Back (\"\")"="Data: Cleanup\nExit") -> ("States Out"=w240:string)  [unwired: 12 in]
        n143 = call <vilib>:"Add State(s) to Queue__JKI_lib_State_Machine.vi"("State(s) in Front (\"\")"=w240, "State(s) in (\"\")"=w243) -> ("States Out"=w242:string)  [unwired: 13 in]
        n144 = Bundle By Name(cluster=w237, "Stop"=FALSE) -> (w235:T10)
      }
      frame "---------- sPanel ----------" {
        # "#CSM \"Category Seperator\"\nDo not put any code in this frame."
      }
      frame "sPanel: Func" {
        w251 = "" ("f")
        n145 = call "Convert API String Arguments to Data.vim"("Reference Type"=cluster{"CSM Name":string, "开关":bool} {"CSM Name"="", "开关"=FALSE} ("簇"), "API String"=w277) -> ("Data"=w273:cluster{"CSM Name":string, "开关":bool})  [unwired: 6 in, 1 out]
        n146 = Unbundle By Name(w272) -> ("索引汇总.子面板索引"=w271:refnum<vi>[], "索引汇总.程序索引"=w270:refnum<vi>[], "索引汇总.开关索引"=w262:refnum<vi>[], "索引汇总.CSM Names"=w261:T9)
        n147 = Unbundle By Name(w273) -> ("CSM Name"=w247:string, "开关"=w257:bool)
        n148 = Search 1D Array(1D array=w261, element=w247) -> (index of element=w254:i32)  [unwired: 1 in]
        n149 = Index Array(array=w271, index=w254) -> (element=w269:refnum<vi>)
        n150 = Index Array(array=w270, index=w254) -> (element=w268:refnum<vi>)
        n151 = Index Array(array=w262, index=w254) -> (element=w263:refnum<vi>)
        n152 = property class="Bool (严格)"(reference=w263, "Value"=w257) -> ()  [unwired: 1 in, 2 out]
        n153 = Search/Split String(string=w247, search string/char (-)="OP" ("搜索字符串/字符(-)")) -> (offset of match=w248:i32)  [unwired: 1 in, 2 out]
        n154 = Less Than 0?(x=w248) -> (x < 0?=w246:bool)
        n155 = Bundle("子面板HM1"=w269, w268, "CSM Name"=w247) -> (w267:T12)  [unwired: 1 in]
        n156 = call "Convert Data To API String Arguments.vim"("Data"=w267) -> ("API String"=w278:string)  [unwired: 7 in, 1 out]
        n157 = Select(t="sPanel: Open", s=w257, f="sPanel: Close") -> (s? t:f=w264:string)
        n158 = Select(t="DSave: Start", s=w257, f="DSave: Stop") -> (s? t:f=w256:string)
        n159 = call <vilib>:"Build State String with Arguments__JKI_lib_State_Machine.vi"("Arguments (\"\")"=w278, "State"=w264) -> ("State with Arguments"=w260:string)  [unwired: 4 in]
        n160 = Select(t=w256, s=w246, f=w251) -> (s? t:f=w255:string)
        n161 = call <vilib>:"Add State(s) to Queue__jki_lib_state_machine.vi"("State(s) in Front (\"\")"=w260, "State(s) in (\"\")"=w255) -> ("States Out"=w252:string)  [unwired: 13 in]
        n162 = Greater Or Equal To 0?(x=w254) -> (x >= 0?=w253:bool)
        n163 = Select(t=w252, s=w253, f=w251) -> (s? t:f=w250:string)
        n164 = call <vilib>:"Add State(s) to Queue__jki_lib_state_machine.vi"("State(s) in Front (\"\")"=w250, "State(s) in (\"\")"=w275) -> ("States Out"=w276:string)  [unwired: 13 in]
      }
      frame "sPanel: Open" {
        # "#CSM API Example\nCopy/Rename this case for your own API"
        n165 = call "Convert API String Arguments to Data.vim"("Reference Type"=T5 {"子面板"=refnum, "程序引用"=refnum, "CSM Name"=""} ("簇"), "API String"=w292) -> ("Data"=w291:T5)  [unwired: 6 in, 1 out]
        n166 = Unbundle(w291) -> ("子面板"=w290:refnum<vi>, "程序引用"=w287:refnum<vi>, "CSM Name"=w286:string)
        n167 = Search/Split String(string=w286, search string/char (-)="OP" ("搜索字符串/字符(-)")) -> (offset of match=w284:i32)  [unwired: 1 in, 2 out]
        n168 = call "打开引用CSM.vi"("子程序？"=TRUE, "引用"=w290, "CSM Name"=w286, "VI"=w287) -> ("错误输出"=w293:errorcluster)  [unwired: 6 in, 1 out]
        n169 = Less Than 0?(x=w284) -> (x < 0?=w282:bool)
        n170 = flat-sequence {
          tunnel: [w299] -> w283
          tunnel: w293 -> [_]
          tunnel: w286 -> [w297]
          frame #0 {
            w300 = "Acquired Data@Acquisition - <1> >> Coll: <1> @Data Collection -><register>"  # Acquired Data@Acquisition - <1> >> Coll: <1> @Data Collection -><register>
            n171 = Wait (ms)(milliseconds to wait=u32 100 ("等待时间（毫秒）")) -> ()  [unwired: 1 out]
            n172 = call <vilib>:"Add State(s) to Queue__JKI_lib_State_Machine.vi"("State(s) in (\"\")"=w300) -> ("States Out"=w301:string)  [unwired: 14 in]
            n173 = call-poly <userlib>:"Build Message with Arguments++.vi"("States With Replace Token"=w301, "<1>"=w297) -> ("States"=w299:string)  [unwired: 13 in]
          }
        }
        n174 = Select(t=w283, s=w282, f="") -> (s? t:f=w280:string)
        n175 = call <vilib>:"Add State(s) to Queue__JKI_lib_State_Machine.vi"("State(s) in Front (\"\")"=w280, "State(s) in (\"\")"=w294) -> ("States Out"=w295:string)  [unwired: 13 in]
      }
      frame "sPanel: Close" {
        w304 = "Acquired Data@Acquisition - <1> >> Coll: <1> @Data Collection -><unregister>"  # Acquired Data@Acquisition - <1> >> Coll: <1> @Data Collection -><unregister>
        n176 = call "Convert API String Arguments to Data.vim"("Reference Type"=T5 {"子面板"=refnum, "程序引用"=refnum, "CSM Name"=""} ("簇"), "API String"=w309) -> ("Data"=w311:T5)  [unwired: 6 in, 1 out]
        n177 = Unbundle By Name(w311) -> ("CSM Name"=w306:string)
        n178 = Search/Split String(string=w306, search string/char (-)="OP" ("搜索字符串/字符(-)")) -> (offset of match=w307:i32)  [unwired: 1 in, 2 out]
        n179 = Less Than 0?(x=w307) -> (x < 0?=w305:bool)
        n180 = Select(t=w304, s=w305, f="") -> (s? t:f=w302:string)
        n181 = call <vilib>:"Build State String with Arguments__JKI_lib_State_Machine.vi"("Arguments (\"\")"=w309, "State"="sPanel: Remove" ("State(s) at Back (\"\")")) -> ("State with Arguments"=w315:string)  [unwired: 4 in]
        n182 = call <vilib>:"Add State(s) to Queue__JKI_lib_State_Machine.vi"("State(s) in Front (\"\")"=w302, "State(s) in (\"\")"="Macro: Exit-@<1>", "State(s) at Back (\"\")"=w315) -> ("States Out"=w314:string)  [unwired: 12 in]
        n183 = call-poly <userlib>:"Build Message with Arguments++.vi"("States With Replace Token"=w314, "<1>"=w306) -> ("States"=w313:string)  [unwired: 13 in]
        n184 = call <vilib>:"Add State(s) to Queue__JKI_lib_State_Machine.vi"("State(s) in Front (\"\")"=w313, "State(s) in (\"\")"=w317) -> ("States Out"=w318:string)  [unwired: 13 in]
      }
      frame "sPanel: Remove" {
        # "#CSM API Example\nCopy/Rename this case for your own API"
        n185 = call "Convert API String Arguments to Data.vim"("Reference Type"=T5 {"子面板"=refnum, "程序引用"=refnum, "CSM Name"=""} ("簇"), "API String"=w327) -> ("Data"=w328:T5)  [unwired: 6 in, 1 out]
        n186 = Unbundle By Name(w324) -> ("Stop"=w323:bool)
        n187 = Unbundle By Name(w328) -> ("程序引用"=w325:refnum<vi>, "子面板"=w326:refnum<vi>)
        n188 = case shown="True" w323 {
          tunnel: [_ w333] -> w330
          tunnel: w326 -> [_ w332]
          frame False {
          }
          frame True {
            n189 = invoke class="SubPnl" method="Remove VI"(reference=w332) -> (error out=w333:errorcluster)  [unwired: 2 in, 2 out]
          }
        }
        n190 = call "Stall Data Flow.vim"("value in"=w325, "milliseconds to wait"=u32 100) -> ("value out"=w322:refnum<vi>)  [unwired: 1 out]
        n191 = call "关闭引用CSM.vi"("错误输入（无错误）"=w330, "引用"=w322) -> ()  [unwired: 9 in, 1 out]
      }
      frame "---------- DSave ----------" {
        n192 = call <vilib>:"Add State(s) to Queue__jki_lib_state_machine.vi"("State(s) in (\"\")"=w334) -> ("States Out"=w335:string)  [unwired: 14 in]
      }
      frame "DSave: Start" {
        n193 = Unbundle By Name(w339) -> ("Data Save"=w340:bool)
        n194 = case shown="False" w340 {
          tunnel: [w348 ""] -> w341
          tunnel: w339 -> [w356 w358]
          tunnel: [w355 w358] -> w338
          frame False {
            w347 = path "D:/sunrise/data"  # 保存路径
            n195 = Bundle By Name(cluster=w356, "Data Save"=TRUE) -> (w355:T10)
            n196 = Bundle(cluster=T6 {"温度保存-时间"="", "合并保存？"=FALSE, "保存路径"=path "D:/sunrise/data", "Intervals"=0.0} ("输出簇"), "温度保存-时间"="温度数据保存文件-时间", "合并保存？"="合并保存？", "保存路径"=w347, "Intervals"=0.5) -> (w351:T6)
            n197 = call "Convert Data To API String Arguments.vim"("Data"=w351) -> ("API String"=w350:string)  [unwired: 7 in, 1 out]
            n198 = call-poly <userlib>:"Build Message with Arguments++.vi"("States With Replace Token"="API: Start >> <param> -@Data Collection", "<param>"=w350) -> ("States"=w348:string)  [unwired: 13 in]
          }
          frame True {
          }
        }
        n199 = call <vilib>:"Add State(s) to Queue__jki_lib_state_machine.vi"("State(s) in Front (\"\")"=w341, "State(s) in (\"\")"=w342) -> ("States Out"=w343:string)  [unwired: 13 in]
      }
      frame "DSave: Stop" {
        n200 = control-ref of="TP1"() -> (w367:refnum<vi>)
        n201 = control-ref of="TP2"() -> (w368:refnum<vi>)
        n202 = control-ref of="WK1"() -> (w369:refnum<vi>)
        n203 = control-ref of="WK2"() -> (w370:refnum<vi>)
        n204 = control-ref of="PS1"() -> (w371:refnum<vi>)
        n205 = control-ref of="PS2"() -> (w372:refnum<vi>)
        n206 = control-ref of="ZO1"() -> (w373:refnum<vi>)
        n207 = control-ref of="MO1"() -> (w374:refnum<vi>)
        n208 = control-ref of="MO2"() -> (w375:refnum<vi>)
        n209 = control-ref of="HM1"() -> (w376:refnum<vi>)
        n210 = control-ref of="DS1"() -> (w377:refnum<vi>)
        n211 = Build Array(w367, w368, w369, w370, w371, w372, w373, w374, w375, w376, w377) -> (w366:refnum<vi>[])
        n212 = for {
          tunnel: w366 -> [w382] mode=indexing
          tunnel: [w381] -> w365 mode=indexing
          n213 = property class="Bool (严格)"(reference=w382) -> ("Value"=w381:bool)  [unwired: 1 in, 2 out]
        }
        n214 = Or Array Elements(Boolean array=w365) -> (logical OR=w361:bool)
        n215 = Bundle By Name(cluster=w360, "Data Save"=w361) -> (w359:T10)
        n216 = Select(t="", s=w361, f="API: Stop -@Data Collection") -> (s? t:f=w364:string)
        n217 = call <vilib>:"Add State(s) to Queue__jki_lib_state_machine.vi"("State(s) in Front (\"\")"=w364, "State(s) in (\"\")"=w378) -> ("States Out"=w379:string)  [unwired: 13 in]
      }
    }
  }
  n218 = while {
    shift-right: [w393] -> _
    shift-left: enum16{"Idle", "Initialize", "Exit"}."Initialize" -> [w394]
    tunnel: "CSM Name" -> [w391]
    shift-right: [w389] -> _
    shift-left: w25 -> [w390]
    shift-right: [w387] -> _
    shift-left: -1 -> [w388]
    shift-right: [w386] -> _
    shift-left: _ -> [w385]
    shift-right: [w384] -> _
    shift-left: _ -> [w383]
    stop <- w392 stop-if-true
    n219 = case shown="\"Idle\", 默认" w394 {
      tunnel: [enum16{"Idle", "Initialize", "Exit"}."Idle" w412 enum16{"Idle", "Initialize", "Exit"}."Exit"] -> w393
      tunnel: [_ _ TRUE] -> w392
      tunnel: w391 -> [w398 w411 _]
      tunnel: w390 -> [w401 w409 w594]
      tunnel: [w401 w410 w594] -> w389
      tunnel: w388 -> [_ w407 _]
      tunnel: [-1 w408 _] -> w387
      tunnel: [w397 w405 _] -> w386
      tunnel: w385 -> [_ w406 w593]
      tunnel: [w395 w403 w591] -> w384
      tunnel: w383 -> [_ w404 w591]
      frame "Initialize" {
        w396 = FALSE  # your data
        n220 = call <userlib>:"CSM - Module Exit Event.vi"("Name (\"\" to Use UUID) In"=w398) -> ("CSM Exit Event"=w399:refnum<user-event>)  [unwired: 8 in, 2 out]
        n221 = register-events(w399) -> (reference out=w397:refnum<event-registration>)  [unwired: 2 in, 1 out]
        n222 = Bundle("your data"=w396) -> (w395:cluster{"your data":bool})  [unwired: 1 in]
      }
      frame "Idle", Default {
        n223 = event shown="[2] 前面板关闭？" {
          selector: w406 -> [_ _ _ _ _ _ _ _ _ _ _ _]
          dyn-events: [_ _ _ _ _ _ _ _ _ _ _ _] -> w405
          timeout: w407 -> [_ _ _ _ _ _ _ _ _ _ _ _]
          tunnel: [_ _ _ enum16{"Idle", "Initialize", "Exit"}."Exit" _ _ _ _ _ _ _ _] -> w412
          tunnel: w411 -> [w414 _ _ _ _ _ _ _ _ _ _ _]
          tunnel: w409 -> [w417 w423 w430 w438 w451 w470 w489 w508 w527 w546 w565 w584]
          tunnel: [w415 w424 w429 w438 w452 w471 w490 w509 w528 w547 w566 w585] -> w410
          tunnel: [-1 _ _ _ _ _ _ _ _ _ _ _] -> w408
          tunnel: w404 -> [w413 w426 w435 w436 w453 w472 w491 w510 w529 w548 w567 w586]
          tunnel: [w413 w426 w435 w436 w453 w472 w491 w510 w529 w548 w567 w586] -> w403
          event Timeout {
            n224 = event-data() -> ()  [unwired: 1 in, 3 out]
            n225 = call-poly <userlib>:"CSM - Filter JKISM String Queue.vi"("States In"=w417) -> ("States Out"=w416:string)  [unwired: 14 in]
            n226 = call <userlib>:"CSM - Forward UI Operations to CSM.vi"("Name (\"\" to Use UUID)"=w414, "State(s) In (\"\")"=w416) -> ("States Out"=w415:string)  [unwired: 8 in, 1 out]
          }
          event "停止": Value Change {
            n227 = event-data() -> ()  [unwired: 1 in, 1 out]
            n228 = Two Button Dialog(message="确定关闭整个程序？" ("消息")) -> (T button?=w421:bool)  [unwired: 2 in]
            n229 = Select(t="Macro: Exit" ("State(s) in Front (\"\")"), s=w421, f="") -> (s? t:f=w419:string)
            n230 = call <vilib>:"Add State(s) to Queue__JKI_lib_State_Machine.vi"("State(s) in Front (\"\")"=w419, "State(s) in (\"\")"=w423) -> ("States Out"=w424:string)  [unwired: 13 in]
          }
          event Panel Close? {
            n231 = event-data() -> ()  [unwired: 1 in, 1 out]
            n232 = Two Button Dialog(message="确定关闭整个程序？" ("消息")) -> (T button?=w428:bool)  [unwired: 2 in]
            n233 = Not(x=w428) -> (.not. x?=w427:bool)
            n234 = Select(t="Macro: Exit" ("State(s) in Front (\"\")"), s=w428, f="") -> (s? t:f=w431:string)
            n235 = call <vilib>:"Add State(s) to Queue__JKI_lib_State_Machine.vi"("State(s) in Front (\"\")"=w431, "State(s) in (\"\")"=w430) -> ("States Out"=w429:string)  [unwired: 13 in]
            n236 = event-data("Discard?"=w427) -> ()  [unwired: 1 in, 1 out]
          }
          event User Event {
            n237 = event-data() -> ()  [unwired: 1 in, 1 out]
          }
          event "OP1": Value Change {
            n238 = event-data() -> ("CtlRef"=w442:refnum<vi>)  [unwired: 1 in, 2 out]
            n239 = property class="Bool (严格)"(reference=w442) -> ("Label.Text"=w440:string)  [unwired: 1 in, 2 out]
            n240 = case shown="False" "OP1" {
              selector: "OP1" -> [_ w457]
              tunnel: [w455 w457] -> w441
              tunnel: [w454 w457] -> w445
              frame False {
                n241 = Two Button Dialog(message="确定关闭？" ("消息")) -> (T button?=w454:bool)  [unwired: 2 in]
                n242 = Not(x=w454) -> (.not. x?=w455:bool)
              }
              frame True {
              }
            }
            n243 = Bundle("Label.Text"=w440, "OP1"="OP1") -> (w444:cluster{"Label.Text":string, "OP1":bool})  [unwired: 1 in]
            n244 = call "Convert Data To API String Arguments.vim"("No Tag Mode? (F)"=TRUE, "Data"=w444) -> ("API String"=w448:string)  [unwired: 6 in, 1 out]
            n245 = property class="Bool (严格)"(reference=w442, "Value"=w441) -> ()  [unwired: 1 in, 2 out]
            n246 = call <vilib>:"Build State String with Arguments__JKI_lib_State_Machine.vi"("Arguments (\"\")"=w448, "State"="sPanel: Func" ("State(s) in Front (\"\")")) -> ("State with Arguments"=w447:string)  [unwired: 4 in]
            n247 = Select(t=w447, s=w445, f="") -> (s? t:f=w450:string)
            n248 = call <vilib>:"Add State(s) to Queue__JKI_lib_State_Machine.vi"("State(s) in Front (\"\")"=w450, "State(s) in (\"\")"=w451) -> ("States Out"=w452:string)  [unwired: 13 in]
          }
          event "TP1": Value Change {
            n249 = event-data() -> ("CtlRef"=w460:refnum<vi>)  [unwired: 1 in, 2 out]
            n250 = property class="Bool (严格)"(reference=w460) -> ("Label.Text"=w459:string)  [unwired: 1 in, 2 out]
            n251 = case shown="False" "TP1" {
              selector: "TP1" -> [_ w476]
              tunnel: [w474 w476] -> w461
              tunnel: [w473 w476] -> w464
              frame False {
                n252 = Two Button Dialog(message="确定关闭？" ("消息")) -> (T button?=w473:bool)  [unwired: 2 in]
                n253 = Not(x=w473) -> (.not. x?=w474:bool)
              }
              frame True {
              }
            }
            n254 = Bundle("Label.Text"=w459, "TP1"="TP1") -> (w463:cluster{"Label.Text":string, "TP1":bool})  [unwired: 1 in]
            n255 = call "Convert Data To API String Arguments.vim"("No Tag Mode? (F)"=TRUE, "Data"=w463) -> ("API String"=w467:string)  [unwired: 6 in, 1 out]
            n256 = property class="Bool (严格)"(reference=w460, "Value"=w461) -> ()  [unwired: 1 in, 2 out]
            n257 = call <vilib>:"Build State String with Arguments__JKI_lib_State_Machine.vi"("Arguments (\"\")"=w467, "State"="sPanel: Func" ("State(s) in Front (\"\")")) -> ("State with Arguments"=w466:string)  [unwired: 4 in]
            n258 = Select(t=w466, s=w464, f="") -> (s? t:f=w469:string)
            n259 = call <vilib>:"Add State(s) to Queue__JKI_lib_State_Machine.vi"("State(s) in Front (\"\")"=w469, "State(s) in (\"\")"=w470) -> ("States Out"=w471:string)  [unwired: 13 in]
          }
          event "WK1": Value Change {
            n260 = event-data() -> ("CtlRef"=w479:refnum<vi>)  [unwired: 1 in, 2 out]
            n261 = property class="Bool (严格)"(reference=w479) -> ("Label.Text"=w478:string)  [unwired: 1 in, 2 out]
            n262 = case shown="False" "WK1" {
              selector: "WK1" -> [_ w495]
              tunnel: [w493 w495] -> w480
              tunnel: [w492 w495] -> w485
              frame False {
                n263 = Two Button Dialog(message="确定关闭？" ("消息")) -> (T button?=w492:bool)  [unwired: 2 in]
                n264 = Not(x=w492) -> (.not. x?=w493:bool)
              }
              frame True {
              }
            }
            n265 = Bundle("Label.Text"=w478, "WK1"="WK1") -> (w484:cluster{"Label.Text":string, "WK1":bool})  [unwired: 1 in]
            n266 = call "Convert Data To API String Arguments.vim"("No Tag Mode? (F)"=TRUE, "Data"=w484) -> ("API String"=w483:string)  [unwired: 6 in, 1 out]
            n267 = property class="Bool (严格)"(reference=w479, "Value"=w480) -> ()  [unwired: 1 in, 2 out]
            n268 = call <vilib>:"Build State String with Arguments__JKI_lib_State_Machine.vi"("Arguments (\"\")"=w483, "State"="sPanel: Func" ("State(s) in Front (\"\")")) -> ("State with Arguments"=w481:string)  [unwired: 4 in]
            n269 = Select(t=w481, s=w485, f="") -> (s? t:f=w488:string)
            n270 = call <vilib>:"Add State(s) to Queue__JKI_lib_State_Machine.vi"("State(s) in Front (\"\")"=w488, "State(s) in (\"\")"=w489) -> ("States Out"=w490:string)  [unwired: 13 in]
          }
          event "PS1": Value Change {
            n271 = event-data() -> ("CtlRef"=w498:refnum<vi>)  [unwired: 1 in, 2 out]
            n272 = property class="Bool (严格)"(reference=w498) -> ("Label.Text"=w499:string)  [unwired: 1 in, 2 out]
            n273 = case shown="False" "PS1" {
              selector: "PS1" -> [_ w514]
              tunnel: [w512 w514] -> w497
              tunnel: [w511 w514] -> w505
              frame False {
                n274 = Two Button Dialog(message="确定关闭？" ("消息")) -> (T button?=w511:bool)  [unwired: 2 in]
                n275 = Not(x=w511) -> (.not. x?=w512:bool)
              }
              frame True {
              }
            }
            n276 = Bundle("Label.Text"=w499, "PS1"="PS1") -> (w504:cluster{"Label.Text":string, "PS1":bool})  [unwired: 1 in]
            n277 = call "Convert Data To API String Arguments.vim"("No Tag Mode? (F)"=TRUE, "Data"=w504) -> ("API String"=w503:string)  [unwired: 6 in, 1 out]
            n278 = call <vilib>:"Build State String with Arguments__JKI_lib_State_Machine.vi"("Arguments (\"\")"=w503, "State"="sPanel: Func" ("State(s) in Front (\"\")")) -> ("State with Arguments"=w501:string)  [unwired: 4 in]
            n279 = property class="Bool (严格)"(reference=w498, "Value"=w497) -> ()  [unwired: 1 in, 2 out]
            n280 = Select(t=w501, s=w505, f="") -> (s? t:f=w507:string)
            n281 = call <vilib>:"Add State(s) to Queue__JKI_lib_State_Machine.vi"("State(s) in Front (\"\")"=w507, "State(s) in (\"\")"=w508) -> ("States Out"=w509:string)  [unwired: 13 in]
          }
          event "ZO1": Value Change {
            n282 = event-data() -> ("CtlRef"=w517:refnum<vi>)  [unwired: 1 in, 2 out]
            n283 = property class="Bool (严格)"(reference=w517) -> ("Label.Text"=w518:string)  [unwired: 1 in, 2 out]
            n284 = case shown="False" "ZO1" {
              selector: "ZO1" -> [_ w533]
              tunnel: [w531 w533] -> w516
              tunnel: [w530 w533] -> w524
              frame False {
                n285 = Two Button Dialog(message="确定关闭？" ("消息")) -> (T button?=w530:bool)  [unwired: 2 in]
                n286 = Not(x=w530) -> (.not. x?=w531:bool)
              }
              frame True {
              }
            }
            n287 = Bundle("Label.Text"=w518, "ZO1"="ZO1") -> (w523:cluster{"Label.Text":string, "ZO1":bool})  [unwired: 1 in]
            n288 = call "Convert Data To API String Arguments.vim"("No Tag Mode? (F)"=TRUE, "Data"=w523) -> ("API String"=w522:string)  [unwired: 6 in, 1 out]
            n289 = call <vilib>:"Build State String with Arguments__JKI_lib_State_Machine.vi"("Arguments (\"\")"=w522, "State"="sPanel: Func" ("State(s) in Front (\"\")")) -> ("State with Arguments"=w520:string)  [unwired: 4 in]
            n290 = property class="Bool (严格)"(reference=w517, "Value"=w516) -> ()  [unwired: 1 in, 2 out]
            n291 = Select(t=w520, s=w524, f="") -> (s? t:f=w526:string)
            n292 = call <vilib>:"Add State(s) to Queue__JKI_lib_State_Machine.vi"("State(s) in Front (\"\")"=w526, "State(s) in (\"\")"=w527) -> ("States Out"=w528:string)  [unwired: 13 in]
          }
          event "MO1": Value Change {
            n293 = event-data() -> ("CtlRef"=w536:refnum<vi>)  [unwired: 1 in, 2 out]
            n294 = property class="Bool (严格)"(reference=w536) -> ("Label.Text"=w538:string)  [unwired: 1 in, 2 out]
            n295 = case shown="False" "MO1" {
              selector: "MO1" -> [_ w552]
              tunnel: [w550 w552] -> w535
              tunnel: [w549 w552] -> w543
              frame False {
                n296 = Two Button Dialog(message="确定关闭？" ("消息")) -> (T button?=w549:bool)  [unwired: 2 in]
                n297 = Not(x=w549) -> (.not. x?=w550:bool)
              }
              frame True {
              }
            }
            n298 = Bundle("Label.Text"=w538, "MO1"="MO1") -> (w542:cluster{"Label.Text":string, "MO1":bool})  [unwired: 1 in]
            n299 = call "Convert Data To API String Arguments.vim"("No Tag Mode? (F)"=TRUE, "Data"=w542) -> ("API String"=w541:string)  [unwired: 6 in, 1 out]
            n300 = call <vilib>:"Build State String with Arguments__JKI_lib_State_Machine.vi"("Arguments (\"\")"=w541, "State"="sPanel: Func" ("State(s) in Front (\"\")")) -> ("State with Arguments"=w539:string)  [unwired: 4 in]
            n301 = property class="Bool (严格)"(reference=w536, "Value"=w535) -> ()  [unwired: 1 in, 2 out]
            n302 = Select(t=w539, s=w543, f="") -> (s? t:f=w545:string)
            n303 = call <vilib>:"Add State(s) to Queue__JKI_lib_State_Machine.vi"("State(s) in Front (\"\")"=w545, "State(s) in (\"\")"=w546) -> ("States Out"=w547:string)  [unwired: 13 in]
          }
          event "HM1": Value Change {
            n304 = event-data() -> ("CtlRef"=w555:refnum<vi>)  [unwired: 1 in, 2 out]
            n305 = property class="Bool (严格)"(reference=w555) -> ("Label.Text"=w556:string)  [unwired: 1 in, 2 out]
            n306 = case shown="False" "HM1" {
              selector: "HM1" -> [_ w571]
              tunnel: [w569 w571] -> w557
              tunnel: [w568 w571] -> w562
              frame False {
                n307 = Two Button Dialog(message="确定关闭？" ("消息")) -> (T button?=w568:bool)  [unwired: 2 in]
                n308 = Not(x=w568) -> (.not. x?=w569:bool)
              }
              frame True {
              }
            }
            n309 = Bundle("Label.Text"=w556, "HM1"="HM1") -> (w561:cluster{"Label.Text":string, "HM1":bool})  [unwired: 1 in]
            n310 = call "Convert Data To API String Arguments.vim"("No Tag Mode? (F)"=TRUE, "Data"=w561) -> ("API String"=w560:string)  [unwired: 6 in, 1 out]
            n311 = property class="Bool (严格)"(reference=w555, "Value"=w557) -> ()  [unwired: 1 in, 2 out]
            n312 = call <vilib>:"Build State String with Arguments__JKI_lib_State_Machine.vi"("Arguments (\"\")"=w560, "State"="sPanel: Func" ("State(s) in Front (\"\")")) -> ("State with Arguments"=w558:string)  [unwired: 4 in]
            n313 = Select(t=w558, s=w562, f="") -> (s? t:f=w564:string)
            n314 = call <vilib>:"Add State(s) to Queue__JKI_lib_State_Machine.vi"("State(s) in Front (\"\")"=w564, "State(s) in (\"\")"=w565) -> ("States Out"=w566:string)  [unwired: 13 in]
          }
          event "DS1": Value Change {
            n315 = event-data() -> ("CtlRef"=w574:refnum<vi>)  [unwired: 1 in, 2 out]
            n316 = property class="Bool (严格)"(reference=w574) -> ("Label.Text"=w575:string)  [unwired: 1 in, 2 out]
            n317 = case shown="False" "DS1" {
              selector: "DS1" -> [_ w590]
              tunnel: [w588 w590] -> w576
              tunnel: [w587 w590] -> w581
              frame False {
                n318 = Two Button Dialog(message="确定关闭？" ("消息")) -> (T button?=w587:bool)  [unwired: 2 in]
                n319 = Not(x=w587) -> (.not. x?=w588:bool)
              }
              frame True {
              }
            }
            n320 = Bundle("Label.Text"=w575, "DS1"="DS1") -> (w580:cluster{"Label.Text":string, "DS1":bool})  [unwired: 1 in]
            n321 = call "Convert Data To API String Arguments.vim"("No Tag Mode? (F)"=TRUE, "Data"=w580) -> ("API String"=w579:string)  [unwired: 6 in, 1 out]
            n322 = property class="Bool (严格)"(reference=w574, "Value"=w576) -> ()  [unwired: 1 in, 2 out]
            n323 = call <vilib>:"Build State String with Arguments__JKI_lib_State_Machine.vi"("Arguments (\"\")"=w579, "State"="sPanel: Func" ("State(s) in Front (\"\")")) -> ("State with Arguments"=w577:string)  [unwired: 4 in]
            n324 = Select(t=w577, s=w581, f="") -> (s? t:f=w583:string)
            n325 = call <vilib>:"Add State(s) to Queue__JKI_lib_State_Machine.vi"("State(s) in Front (\"\")"=w583, "State(s) in (\"\")"=w584) -> ("States Out"=w585:string)  [unwired: 13 in]
          }
        }
      }
      frame "Exit" {
        n326 = Unregister For Events(event registration refnum=w593) -> (error out=w592:errorcluster)  [unwired: 1 in]
        n327 = call <vilib>:"Clear Errors.vi"("error in (no error)"=w592) -> ()  [unwired: 5 in, 2 out]
      }
    }
  }
  n328 = flat-sequence {
    tunnel: w1 -> [_]
    frame #0 {
      n329 = call "Data Collection and Save.vi"("CSM Name"="Data Collection") -> ()  [unwired: 11 in]
    }
  }
  n330 = call <userlib>:"CSM - Sync Configuration Variables to File.vi"("All Temp Variable to Default Ini(F)"=TRUE, "error in (no error)"=w7) -> ()  [unwired: 7 in, 1 out]
